vi "GDSProject_GuessFolderPath.vi"(1 "ProjectItem":refnum<vi>, 5 "error in (no error)":errorcluster) -> (15 "Path":path, 16 "FoldersToCreate":string, 17 "FolderScopes":T1(array[ring]), 19 "error out":errorcluster)   [LabVIEW 2020]
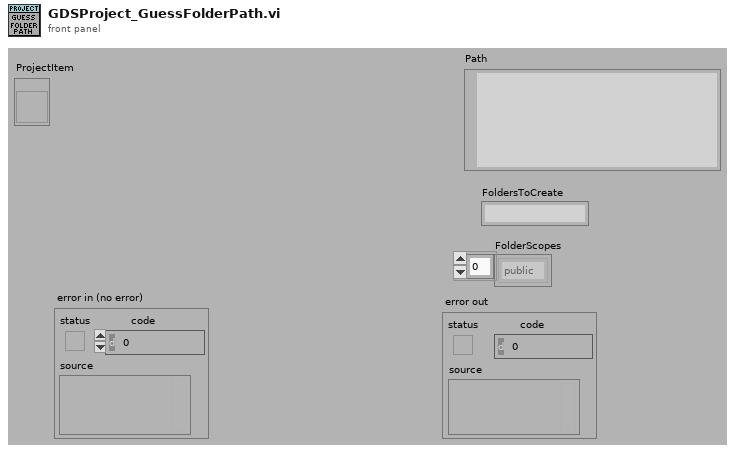
[diagram p1: front panel]
types:
  T1 = enum32{"invalid scope", "public", "private", "protected", "community"}[]
  T2 = enum32{"invalid scope", "public", "private", "protected", "community"}
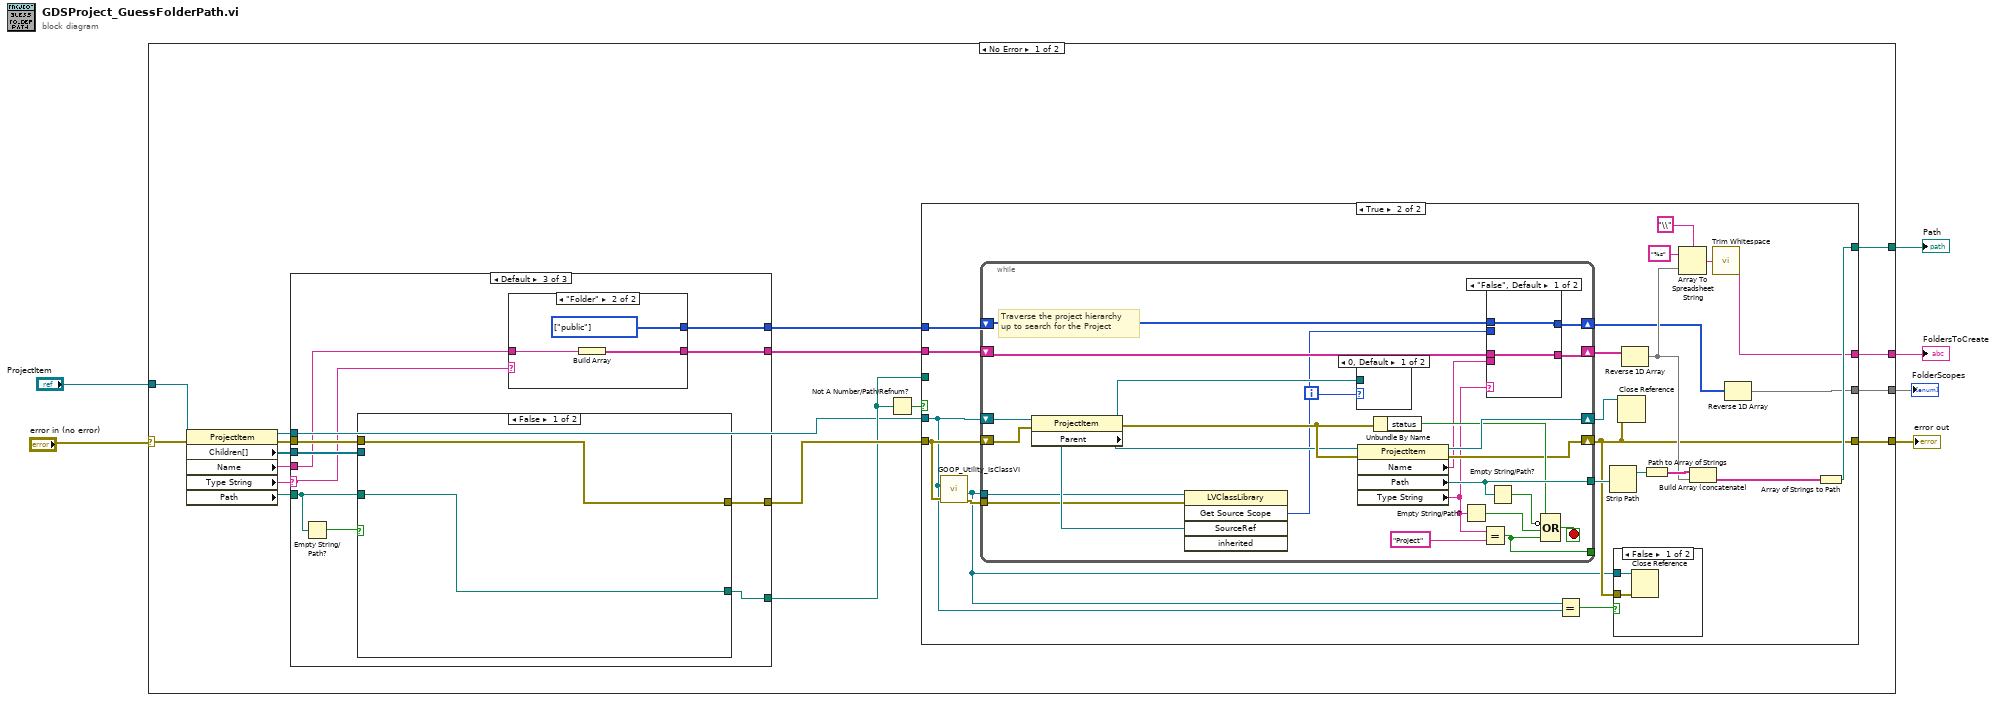
[diagram p0: block diagram]
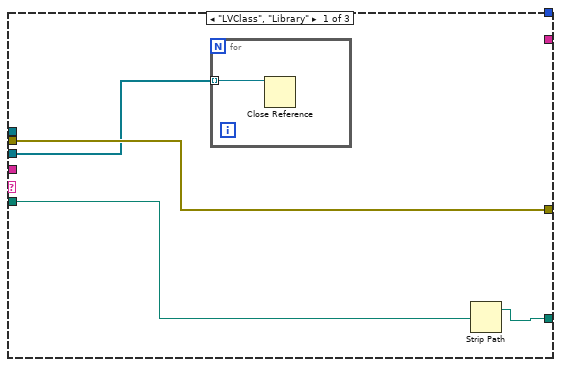
[diagram p2: hidden frame]
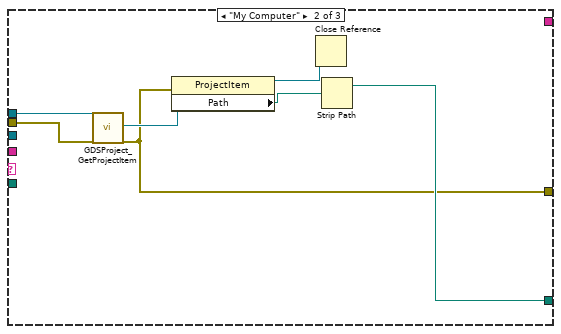
[diagram p3: hidden frame]
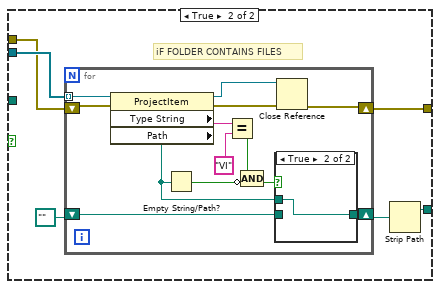
[diagram p4: hidden frame]
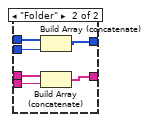
[diagram p9: hidden frame]
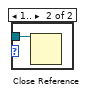
[diagram p10: hidden frame]
diagram:
  n1 = case shown="No Error" "error in (no error)" {
    selector: "error in (no error)" -> [w20 w131]
    tunnel: [w21 w131] -> w5
    tunnel: "ProjectItem" -> [w19 _]
    tunnel: [w22 _] -> w4
    tunnel: [w14 _] -> w3
    tunnel: [w12 _] -> w2
    frame No Error {
      n2 = property class="ProjectItem"(reference=w19, error in=w20) -> (reference out=w7:refnum<vi>, error out=w17:errorcluster, "Children[]"=w18:refnum<vi>[], "Name"=w16:string, "Type String"=w10:string, "Path"=w9:path)
      n3 = case shown="Default" w10 {
        selector: w10 -> [_ _ w39]
        tunnel: w18 -> [w26 _ w45]
        tunnel: [w24 w30 w38] -> w8
        tunnel: w17 -> [w27 w31 w44]
        tunnel: w16 -> [_ _ w43]
        tunnel: [_ _ w42] -> w15
        tunnel: [_ _ w41] -> w13
        tunnel: [w27 w29 w40] -> w11
        tunnel: w9 -> [w25 _ w36]
        tunnel: w7 -> [_ w35 _]
        frame "LVClass", "Library" {
          n4 = for {
            tunnel: w26 -> [w28] mode=indexing
            n5 = Close Reference(reference=w28) -> ()  [unwired: 1 in, 1 out]
          }
          n6 = Strip Path(path=w25) -> (stripped path=w24:path)  [unwired: 1 out]
        }
        frame "My Computer" {
          n7 = call "GDSProject_GetProjectItem.vi"("ProjectItemToSearchFrom"=w35, "error in (no error)"=w31) -> ("ProjectItemFound"=w32:refnum<vi>, "error out"=w29:errorcluster)  [unwired: 14 in, 2 out]
          n8 = property class="ProjectItem"(reference=w32, error in=w29) -> (reference out=w34:refnum<vi>, "Path"=w33:path)  [unwired: 1 out]
          n9 = Close Reference(reference=w34) -> ()  [unwired: 1 in, 1 out]
          n10 = Strip Path(path=w33) -> (stripped path=w30:path)  [unwired: 1 out]
        }
        frame Default {
          n11 = Empty String/Path?(string/path=w36) -> (empty?=w37:bool)
          n12 = case shown="False" w37 {
            tunnel: w45 -> [_ w53]
            tunnel: w44 -> [w46 w51]
            tunnel: [w46 w50] -> w40
            tunnel: [w47 w48] -> w38
            tunnel: w36 -> [w47 _]
            frame False {
            }
            frame True {
              # "iF FOLDER CONTAINS FILES"
              n13 = for {
                shift-right: [w60] -> w50
                shift-left: w51 -> [w66]
                tunnel: w53 -> [w65] mode=indexing
                shift-right: [w63] -> w49
                shift-left: path "" ("Path") -> [w64]
                n14 = property class="ProjectItem"(reference=w65, error in=w66) -> (reference out=w62:refnum<vi>, error out=w61:errorcluster, "Type String"=w55:string, "Path"=w59:path)
                n15 = Empty String/Path?(string/path=w59) -> (empty?=w58:bool)
                n16 = Equal?(x=w55, y="VI") -> (x = y?=w56:bool)
                n17 = Compound Arithmetic op=AND(w56, invert w58) -> (w57:bool)
                n18 = case shown="True" w57 {
                  tunnel: w64 -> [w67 _]
                  tunnel: [w67 w68] -> w63
                  tunnel: w59 -> [_ w68]
                  frame False {
                  }
                  frame True {
                  }
                }
                n19 = Close Reference(reference=w62, error in (no error)=w61) -> (error out=w60:errorcluster)
              }
              n20 = Strip Path(path=w49) -> (stripped path=w48:path)  [unwired: 1 out]
            }
          }
          n21 = case shown="\"Folder\"" w39 {
            tunnel: w43 -> [_ w71]
            tunnel: [_ w70] -> w42
            tunnel: [_ w69] -> w41
            frame Default {
            }
            frame "Folder" {
              w69 = T1 [enum."public"] items=["invalid scope", "public", "private", "protected", "community"]
              n22 = Build Array(w71) -> (w70:string[])
            }
          }
        }
      }
      n23 = Not A Number/Path/Refnum?(number/path/refnum=w8) -> (NaN/Path/Refnum?=w23:bool)
      n24 = case shown="True" w23 {
        tunnel: w11 -> [w72 w78]
        tunnel: w7 -> [_ w76]
        tunnel: [w73 w94] -> w22
        tunnel: w8 -> [w73 _]
        tunnel: [w72 w79] -> w21
        tunnel: w15 -> [_ w89]
        tunnel: [_ w82] -> w14
        tunnel: w13 -> [_ w84]
        tunnel: [_ w80] -> w12
        frame False {
        }
        frame True {
          n25 = call "GOOP_Utility_IsClassVI.vi"("error in (no error)"=w78, "ProjectItem"=w76) -> ("error out"=w77:errorcluster, "ClassItem(If Found)"=w75:refnum<vi>)  [unwired: 4 in, 4 out]
          n26 = while {
            shift-right: [w120] -> w90
            shift-left: w76 -> [w121]
            tunnel: [w113] -> w92
            tunnel: [w114] -> _
            shift-right: [w109] -> w79
            shift-left: w78 -> [w103]
            shift-right: [w106] -> w88
            shift-left: w89 -> [w107]
            shift-right: [w101] -> w81
            shift-left: w84 -> [w100]
            tunnel: w75 -> [w99]
            tunnel: w77 -> [w98]
            i -> [w116]
            stop <- w119 stop-if-true
            # "Traverse the project hierarchy\nup to search for the Project"
            n27 = property class="ProjectItem"(reference=w121, error in=w103) -> (reference out=w117:refnum<vi>, error out=w110:errorcluster, "Parent"=w104:refnum<vi>)
            n28 = invoke class="LVClassLibrary" method="Get Source Scope"(reference=w99, error in=w98, "SourceRef"=w104) -> ("GetSourceScope"=w102:T2)  [unwired: 2 in, 4 out]
            n29 = case shown="0, Default" w116 {
              tunnel: w117 -> [_ w130]
              frame 0, Default {
              }
              frame 1.. {
                n30 = Close Reference(reference=w130) -> ()  [unwired: 1 in, 1 out]
              }
            }
            n31 = property class="ProjectItem"(reference=w104, error in=w110) -> (reference out=w120:refnum<vi>, error out=w109:errorcluster, "Name"=w105:string, "Path"=w113:path, "Type String"=w108:string)
            n32 = Unbundle By Name(w110) -> ("status"=w112:bool)
            n33 = Empty String/Path?(string/path=w108) -> (empty?=w115:bool)
            n34 = Equal?(x=w108, y="Project") -> (x = y?=w114:bool)
            n35 = case shown="\"False\", Default" w108 {
              tunnel: w107 -> [w123 w129]
              tunnel: [w123 w128] -> w106
              tunnel: w105 -> [_ w127]
              tunnel: w102 -> [_ w126]
              tunnel: [w122 w125] -> w101
              tunnel: w100 -> [w122 w124]
              frame "False", Default {
              }
              frame "Folder" {
                n36 = Build Array (concatenate)(w124, w126) -> (w125:T1)
                n37 = Build Array (concatenate)(w129, w127) -> (w128:string[])
              }
            }
            n38 = Empty String/Path?(string/path=w113) -> (empty?=w111:bool)
            n39 = Compound Arithmetic op=OR(w112, invert w111, w115, w114) -> (w119:bool)
          }
          n40 = Equal?(x=w75, y=w76) -> (x = y?=w74:bool)
          n41 = Strip Path(path=w92) -> (stripped path=w91:path)  [unwired: 1 out]
          n42 = case shown="False" w74 {
            tunnel: w79 -> [w97 _]
            tunnel: w75 -> [w96 _]
            frame False {
              n43 = Close Reference(reference=w96, error in (no error)=w97) -> ()  [unwired: 1 out]
            }
            frame True {
            }
          }
          n44 = Close Reference(reference=w90, error in (no error)=w79) -> ()  [unwired: 1 out]
          n45 = Reverse 1D Array(array=w88) -> (reversed array=w83:string[])
          n46 = Path to Array of Strings(0:w91) -> (2:w95:string[])  [unwired: 1 out]
          n47 = Array To Spreadsheet String(delimiter (Tab)="\\", array=w83, 3:"%s" ("format string")) -> (spreadsheet string=w85:string)
          n48 = Build Array (concatenate)(w95, w83) -> (w93:string[])
          n49 = call <vilib>:"Trim Whitespace.vi"("string"=w85) -> ("trimmed string"=w82:string)  [unwired: 1 in]
          n50 = Reverse 1D Array(array=w81) -> (reversed array=w80:T1)
          n51 = Array of Strings to Path(0:w93) -> (2:w94:path)  [unwired: 1 in]
        }
      }
    }
    frame Error {
    }
  }
  "error out" <- w5
  "Path" <- w4
  "FoldersToCreate" <- w3
  "FolderScopes" <- w2
